vi "Exo_5.1.vi"(11 "N":i32) -> (0 "Array":dbl[](array[numeric]))   [LabVIEW 2012]
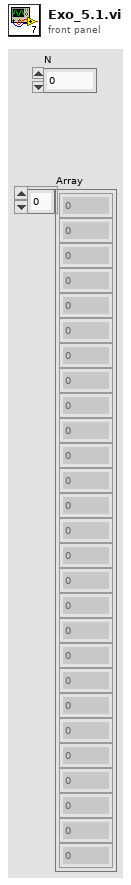
[diagram p1: front panel]
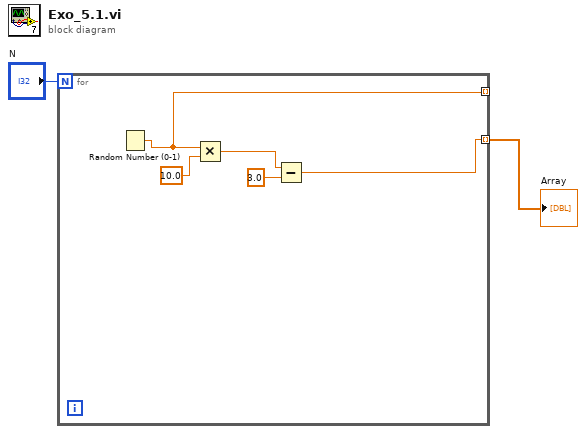
[diagram p0: block diagram]
diagram:
  n1 = for {
    N: "N" -> [_]
    tunnel: [w4] -> w1 mode=indexing
    tunnel: [w3] -> _ mode=indexing
    n2 = Random Number (0-1)() -> (number: 0 to 1=w3:dbl)
    n3 = Multiply(x=w3, y=10.0) -> (x*y=w6:dbl)
    n4 = Subtract(x=w6, y=3.0) -> (x-y=w4:dbl)
  }
  "Array" <- w1
